vi "ConvertTextBasedCodeToLabVIEW_CreateMissingTypeList.vi"(9 "EnumsOusideClass":T1[](array[typedef]), 10 "StructsOusideClass":T4[](array[typedef]), 11 "Classes":T7[](array[typedef])) -> (3 "MissingItems":T13[](array[typedef]))   [LabVIEW 2020]
uses:
  ConvertTextBasedCodeToLabVIEW_MissingType.ctl
  ConvertTextBasedCodeToLabVIEW_MissingTypeIconType.ctl
  String/GDSString_ClassDescriptionType.ctl
  String/GDSString_AccessScopeModifierType.ctl
  String/GDSString_ModifierType.ctl
  String/GDSString_MethodDescriptionType.ctl
  CommonVIs/CommonVIs_AttributeType.ctl
  CommonVIs/CommonVIs_AttributeDataType.ctl
  CommonVIs/CommonVIs_PropertyType.ctl
  String/GDSString_ClassParentType.ctl
  String/GDSString_ClassType.ctl
  String/GDSString_ClassOwnerType.ctl
  CommonVIs/CommonVIs_EnumType.ctl
  CommonVIs/CommonVIs_StructType.ctl
  ConvertTextBasedCodeToLabVIEW_MissingTypeOptions.ctl
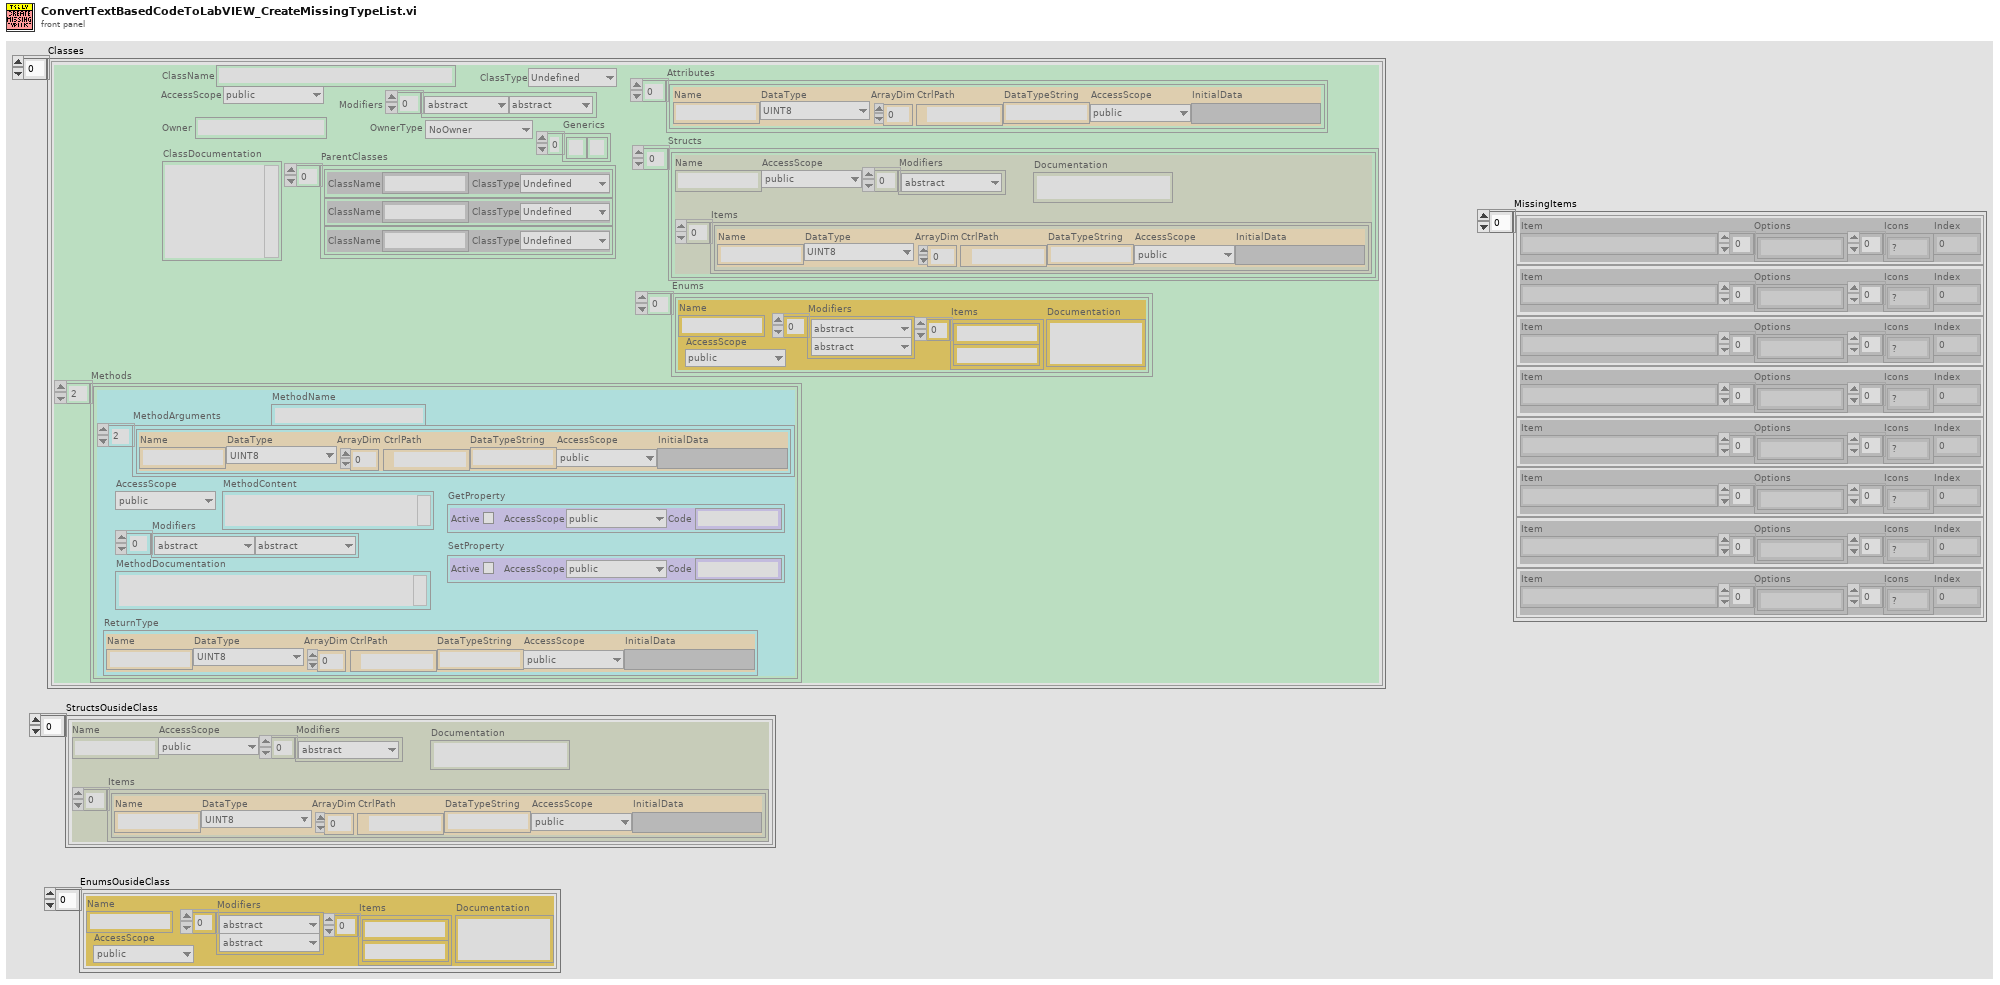
[diagram p1: front panel]
types:
  T1 = typedef "CommonVIs_EnumType.ctl" = cluster{"Name":string, "AccessScope":T2, "Modifiers":T3[], "Items":string[], "Documentation":string}
  T2 = typedef "GDSString_AccessScopeModifierType.ctl" = enum16{"public", "private", "protected", "internal"}
  T3 = typedef "GDSString_ModifierType.ctl" = enum16{"abstract", "static", "final", "synchronized", "strictfp", "async", "const", "event", "extern", "new", "native ", "override", "partial", "readonly", "sealed", "unsafe", "virtual", "volatile"}
  T4 = typedef "CommonVIs_StructType.ctl" = cluster{"Name":string, "AccessScope":T2, "Modifiers":T3[], "Items":T5[], "Documentation":string}
  T5 = typedef "CommonVIs_AttributeType.ctl" = cluster{"Name":string, "DataType":T6, "ArrayDim":i32, "CtrlPath":path, "DataTypeString":string, "AccessScope":T2, "InitialData":variant}
  T6 = typedef "CommonVIs_AttributeDataType.ctl" = enum16{"UINT8", "INT8", "UINT16", "INT16", "UINT32", "INT32", "UINT64", "INT64", "SGL", "DBL", "EXT", "CSG", "CDB", "CXT", "TimeStamp", "STRING", "PATH", "BOOL", "ENUM", "RefNum", "VIRefNum", "LabVIEW Class", "Cluster", "Variant", "TypeDef", "Waveform", "LabVIEW Object", "Other", "void", "Set", "Map"}
  T7 = typedef "GDSString_ClassDescriptionType.ctl" = cluster{"ClassName":string, "AccessScope":T2, "Modifiers":T3[], "ClassDocumentation":string, "Methods":T8[], "ParentClasses":T10[], "ClassType":T11, "Owner":string, "OwnerType":T12, "Generics":string[], "Attributes":T5[], "Enums":T1[], "Structs":T4[]}
  T8 = typedef "GDSString_MethodDescriptionType.ctl" = cluster{"ReturnType":T5, "MethodName":string, "AccessScope":T2, "Modifiers":T3[], "MethodDocumentation":string, "MethodContent":string, "MethodArguments":T5[], "GetProperty":T9, "SetProperty":T9}
  T9 = typedef "CommonVIs_PropertyType.ctl" = cluster{"Active":bool, "AccessScope":T2, "Code":string}
  T10 = typedef "GDSString_ClassParentType.ctl" = cluster{"ClassName":string, "ClassType":T11}
  T11 = typedef "GDSString_ClassType.ctl" = enum16{"Undefined", "Class", "Interface"}
  T12 = typedef "GDSString_ClassOwnerType.ctl" = enum16{"NoOwner", "Class", "Package/NameSpace"}
  T13 = typedef "ConvertTextBasedCodeToLabVIEW_MissingType.ctl" = cluster{"Item":string, "Options":string[], "Icons":T14[], "Index":i32}
  T14 = typedef "ConvertTextBasedCodeToLabVIEW_MissingTypeIconType.ctl" = enum16{"?", "Add", "Delete", "Implement", "Inherit"}
  T15 = typedef "ConvertTextBasedCodeToLabVIEW_MissingTypeOptions.ctl" = enum16{"Select action to handle missing type", "Create stub code as class", "Create stub code as interface", "Remove dependency to this type"}
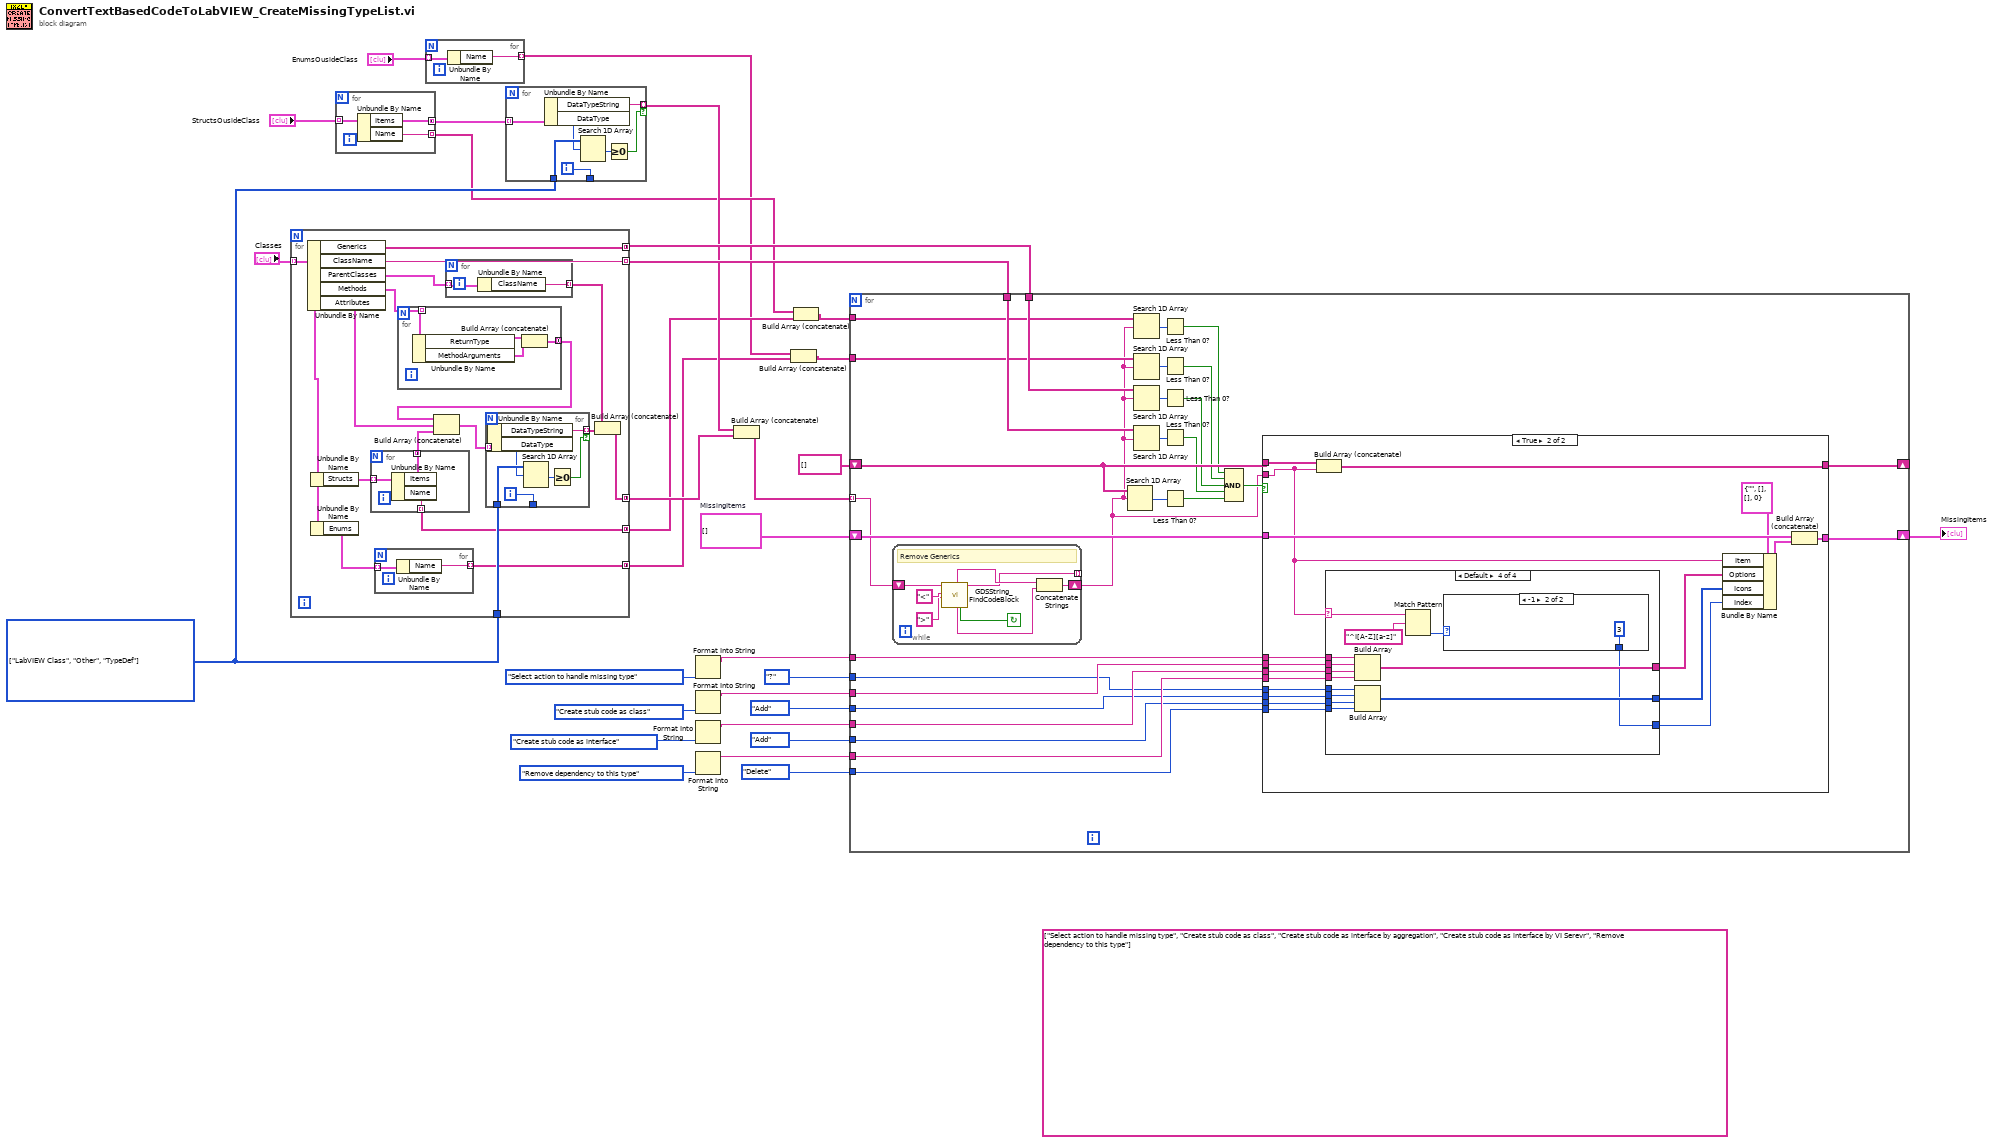
[diagram p0: block diagram]
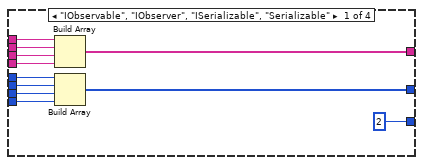
[diagram p3: hidden frame]
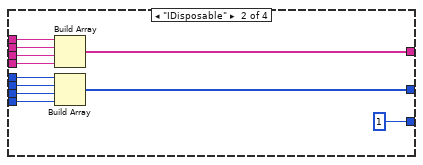
[diagram p4: hidden frame]
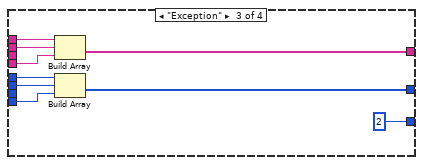
[diagram p5: hidden frame]
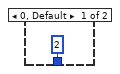
[diagram p6: hidden frame]
diagram:
  (unwired) string[] ["Select action to handle missing type", "Create stub code as class", "Create stub code as interface by aggregation", "Create stub code as interface by VI Serevr", "Remove dependency to this type"] ("Options")
  w27 = T13[] []  # MissingItems
  w10 = T6[] [enum."LabVIEW Class", enum."Other", enum."TypeDef"] items=["UINT8", "INT8", "UINT16", "INT16", "UINT32", "INT32", "UINT64", "INT64", "SGL", "DBL", "EXT", "CSG", "CDB", "CXT", "TimeStamp", "STRING", "PATH", "BOOL", "ENUM", "RefNum", "VIRefNum", "LabVIEW Class", "Cluster", "Variant", "TypeDef", "Waveform", "LabVIEW Object", "Other", "void", "Set", "Map"] ("1D array")
  n1 = for {
    tunnel: "Classes" -> [w34] mode=indexing
    tunnel: [w48] -> w30 mode=indexing
    tunnel: [w36] -> w7 mode=concatenating
    tunnel: w10 -> [w38]
    tunnel: [w44] -> w31 mode=concatenating
    tunnel: [w35] -> w6 mode=concatenating
    tunnel: [w32] -> w3 mode=concatenating
    n2 = Unbundle By Name(w34) -> ("Generics"=w44:string[], "ClassName"=w48:string, "ParentClasses"=w47:T10[], "Methods"=w46:T8[], "Attributes"=w43:T5[])
    n3 = Unbundle By Name(w34) -> ("Structs"=w41:T4[])
    n4 = Unbundle By Name(w34) -> ("Enums"=w33:T1[])
    n5 = for {
      tunnel: w41 -> [w60] mode=indexing
      tunnel: [w59] -> w40 mode=concatenating
      tunnel: [w58] -> w35 mode=indexing
      n6 = Unbundle By Name(w60) -> ("Items"=w59:T5[], "Name"=w58:string)
    }
    n7 = for {
      tunnel: w33 -> [w50] mode=indexing
      tunnel: [w49] -> w32 mode=indexing
      n8 = Unbundle By Name(w50) -> ("Name"=w49:string)
    }
    n9 = for {
      tunnel: w46 -> [w64] mode=indexing
      tunnel: [w61] -> w42 mode=concatenating
      n10 = Unbundle By Name(w64) -> ("ReturnType"=w63:T5, "MethodArguments"=w62:T5[])
      n11 = Build Array (concatenate)(w63, w62) -> (w61:T5[])
    }
    n12 = Build Array (concatenate)(w42, w43, w40) -> (w39:T5[])
    n13 = for {
      tunnel: w47 -> [w66] mode=indexing
      tunnel: [w65] -> w45 mode=indexing
      n14 = Unbundle By Name(w66) -> ("ClassName"=w65:string)
    }
    n15 = for {
      tunnel: w39 -> [w57] mode=indexing
      tunnel: w38 -> [w56]
      tunnel: [w53] -> w37 mode=indexing if=w52
      tunnel: [w51] -> _
      i -> [w51]
      n16 = Unbundle By Name(w57) -> ("DataTypeString"=w53:string, "DataType"=w55:T6)
      n17 = Search 1D Array(1D array=w56, element=w55) -> (index of element=w54:i32)  [unwired: 1 in]
      n18 = Greater Or Equal To 0?(x=w54) -> (x >= 0?=w52:bool)
    }
    n19 = Build Array (concatenate)(w45, w37) -> (w36:string[])
  }
  n20 = for {
    tunnel: "StructsOusideClass" -> [w69] mode=indexing
    tunnel: [w68] -> w11 mode=concatenating
    tunnel: [w67] -> w4 mode=indexing
    n21 = Unbundle By Name(w69) -> ("Items"=w68:T5[], "Name"=w67:string)
  }
  n22 = for {
    tunnel: "EnumsOusideClass" -> [w71] mode=indexing
    tunnel: [w70] -> w1 mode=indexing
    n23 = Unbundle By Name(w71) -> ("Name"=w70:string)
  }
  n24 = for {
    tunnel: w11 -> [w78] mode=indexing
    tunnel: w10 -> [w77]
    tunnel: [w74] -> w9 mode=indexing if=w73
    tunnel: [w72] -> _
    i -> [w72]
    n25 = Unbundle By Name(w78) -> ("DataTypeString"=w74:string, "DataType"=w76:T6)
    n26 = Search 1D Array(1D array=w77, element=w76) -> (index of element=w75:i32)  [unwired: 1 in]
    n27 = Greater Or Equal To 0?(x=w75) -> (x >= 0?=w73:bool)
  }
  n28 = Format Into String(ConvertTextBasedCodeToLabVIEW_MissingTypeOptions."Select action to handle missing type") -> (resulting string=w17:string)  [unwired: 3 in, 1 out]
  n29 = Format Into String(ConvertTextBasedCodeToLabVIEW_MissingTypeOptions."Create stub code as class") -> (resulting string=w14:string)  [unwired: 3 in, 1 out]
  n30 = Format Into String(ConvertTextBasedCodeToLabVIEW_MissingTypeOptions."Create stub code as interface") -> (resulting string=w18:string)  [unwired: 3 in, 1 out]
  n31 = Format Into String(ConvertTextBasedCodeToLabVIEW_MissingTypeOptions."Remove dependency to this type") -> (resulting string=w20:string)  [unwired: 3 in, 1 out]
  n32 = Build Array (concatenate)(w9, w7) -> (w8:string[])
  n33 = Build Array (concatenate)(w1, w3) -> (w2:string[])
  n34 = Build Array (concatenate)(w4, w6) -> (w5:string[])
  n35 = for {
    tunnel: w8 -> [w86] mode=indexing
    shift-right: [w103] -> _
    shift-left: string[] [] -> [w104]
    tunnel: w30 -> [w102]
    tunnel: w31 -> [w99]
    shift-right: [w95] -> w26
    shift-left: w27 -> [w96]
    tunnel: w17 -> [w94]
    tunnel: w14 -> [w93]
    tunnel: w18 -> [w92]
    tunnel: w20 -> [w91]
    tunnel: ConvertTextBasedCodeToLabVIEW_MissingTypeIconType."?" ("Icon") -> [w90]
    tunnel: ConvertTextBasedCodeToLabVIEW_MissingTypeIconType."Add" ("Icon") -> [w89]
    tunnel: ConvertTextBasedCodeToLabVIEW_MissingTypeIconType."Add" ("Icon") -> [w88]
    tunnel: ConvertTextBasedCodeToLabVIEW_MissingTypeIconType."Delete" ("Icon") -> [w87]
    tunnel: w5 -> [w83]
    tunnel: w2 -> [w82]
    n36 = while {
      shift-right: [w109] -> w81
      shift-left: w86 -> [w115]
      tunnel: [w108] -> _ mode=indexing
      stop <- w112 continue-if-true
      # "Remove Generics"
      n37 = call "GDSString_FindCodeBlock.vi"("Text"=w115, "CodeBlockStartCharacter( { )"="<", "CodeBlockEndCharacter( } )"=">") -> ("TextBeforeBlock"=w111:string, "TextAfterBlock"=w110:string, "found"=w112:bool, "BlockText"=w108:string)  [unwired: 8 in, 5 out]
      n38 = Concatenate Strings(w111, w110) -> (w109:string)
    }
    n39 = Search 1D Array(1D array=w104, element=w81) -> (index of element=w107:i32)  [unwired: 1 in]
    n40 = Search 1D Array(1D array=w83, element=w81) -> (index of element=w85:i32)  [unwired: 1 in]
    n41 = Search 1D Array(1D array=w82, element=w81) -> (index of element=w84:i32)  [unwired: 1 in]
    n42 = Search 1D Array(1D array=w99, element=w81) -> (index of element=w98:i32)  [unwired: 1 in]
    n43 = Search 1D Array(1D array=w102, element=w81) -> (index of element=w101:i32)  [unwired: 1 in]
    n44 = Less Than 0?(x=w85) -> (x < 0?=w79:bool)
    n45 = Less Than 0?(x=w84) -> (x < 0?=w80:bool)
    n46 = Less Than 0?(x=w98) -> (x < 0?=w97:bool)
    n47 = Less Than 0?(x=w101) -> (x < 0?=w100:bool)
    n48 = Less Than 0?(x=w107) -> (x < 0?=w105:bool)
    n49 = Compound Arithmetic op=AND(w79, w80, w97, w100, w105) -> (w106:bool)
    n50 = case shown="True" w106 {
      tunnel: w104 -> [w117 w135]
      tunnel: w81 -> [_ w129]
      tunnel: [w117 w134] -> w103
      tunnel: w96 -> [w116 w133]
      tunnel: [w116 w132] -> w95
      tunnel: w94 -> [_ w128]
      tunnel: w93 -> [_ w127]
      tunnel: w92 -> [_ w126]
      tunnel: w91 -> [_ w125]
      tunnel: w90 -> [_ w124]
      tunnel: w89 -> [_ w123]
      tunnel: w88 -> [_ w122]
      tunnel: w87 -> [_ w121]
      frame False {
      }
      frame True {
        n51 = Build Array (concatenate)(w135, w129) -> (w134:string[])
        n52 = case shown="Default" w129 {
          selector: w129 -> [_ _ _ w180]
          tunnel: w128 -> [w146 w157 w166 w177]
          tunnel: w127 -> [w145 w156 w165 w176]
          tunnel: w126 -> [w144 w155 _ w175]
          tunnel: w125 -> [w143 w154 w164 w174]
          tunnel: w124 -> [w142 w153 w163 w170]
          tunnel: w123 -> [w141 w152 w162 w171]
          tunnel: w122 -> [w140 w151 _ w172]
          tunnel: w121 -> [w139 w150 w161 w173]
          tunnel: [w138 w149 w160 w169] -> w120
          tunnel: [w137 w148 w159 w168] -> w119
          tunnel: [2 ("InitialIndex") 1 ("InitialIndex") 2 ("InitialIndex") w167] -> w118
          frame "IObservable", "IObserver", "ISerializable", "Serializable" {
            n53 = Build Array(w146, w145, w144, w143) -> (w138:string[])
            n54 = Build Array(w142, w141, w140, w139) -> (w137:T14[])
          }
          frame "IDisposable" {
            n55 = Build Array(w157, w156, w155, w154) -> (w149:string[])
            n56 = Build Array(w153, w152, w151, w150) -> (w148:T14[])
          }
          frame "Exception" {
            n57 = Build Array(w166, w165, w164) -> (w160:string[])
            n58 = Build Array(w163, w162, w161) -> (w159:T14[])
          }
          frame Default {
            n59 = Build Array(w177, w176, w175, w174) -> (w169:string[])
            n60 = Build Array(w170, w171, w172, w173) -> (w168:T14[])
            n61 = Match Pattern(string=w180, regular expression="^I[A-Z][a-z]") -> (offset past match=w178:i32)  [unwired: 1 in, 3 out]
            n62 = case shown="-1" w178 {
              tunnel: [2 ("InitialIndex") 3 ("InitialIndex")] -> w167
              frame 0, Default {
              }
              frame -1 {
              }
            }
          }
        }
        n63 = Bundle By Name(cluster=T13 {"Item"="", "Options"=[], "Icons"=[], "Index"=0} ("Cluster"), "Item"=w129, "Options"=w120, "Icons"=w119, "Index"=w118) -> (w130:T13)
        n64 = Build Array (concatenate)(w133, w130) -> (w132:T13[])
      }
    }
  }
  "MissingItems" <- w26
